vi "edge_detecting.vi"(0 "Image In":T5=refnum, 1 "mid_near Edge Options":T3={"Edge Polarity"=0, "Kernel Size"=3, "Width"=3, "Minimum Edge Strength"=10.0, "Interpolation Type"=enum."Bilinear Fixed", "Data Processing Method"=enum."Average"} {"Edge Polarity" items=["All Edges", "Rising Edges", "Falling Edges"]}, 2 "mid_far Edge Options":T3={"Edge Polarity"=0, "Kernel Size"=3, "Width"=3, "Minimum Edge Strength"=10.0, "Interpolation Type"=enum."Bilinear Fixed", "Data Processing Method"=enum."Average"} {"Edge Polarity" items=["All Edges", "Rising Edges", "Falling Edges"]}, 4 "mid_near Descriptor":T4={"Global Rectangle"=[276, 216, 344, 218], "Contours"=[{"ID"=enum."External", "Type"=2, "Coordinates"=[276, 216, 343, 217]}]} {"Contours"."Type" items=["No Selection", "Point", "Line", "Rectangle", "Oval", "Polygon", "Freehand Region", "Annulus", "Unused2", "Unused3", "Broken Line", "Freehand Line", "Rotated Rectangle"]}, 5 "mid_far Descriptor":T4={"Global Rectangle"=[475, 215, 533, 216], "Contours"=[{"ID"=enum."External", "Type"=2, "Coordinates"=[475, 215, 532, 215]}]} {"Contours"."Type" items=["No Selection", "Point", "Line", "Rectangle", "Oval", "Polygon", "Freehand Region", "Annulus", "Unused2", "Unused3", "Broken Line", "Freehand Line", "Rotated Rectangle"]}, 7 "error in":errorcluster) -> (20 "Image Out":T5, 21 "mid_near Edge Information":T1[](array[typedef]) {"Distance (Real-World)" format="%.2f"; "Location (Real-World)"."Y" format="%.2g"; "Location (Real-World)"."X" format="%.2f"; "Noise" format="%.2f"; "Location (Pixel)"."Y" format="%.2g"; "Location (Pixel)"."X" format="%.2f"; "Strength" format="%.2f"; "Distance (Pixel)" format="%.2f"}, 22 "mid_far Edge Information":T1[](array[typedef])=[{"Location (Pixel)"={"X"=519.67285, "Y"=215.0}, "Location (Real-World)"={"X"=240.41748, "Y"=115.199524}, "Distance (Pixel)"=44.6728401184082, "Distance (Real-World)"=30.526857895066314, "Strength"=12.0, "Noise"=4.0, "Rising?"=TRUE}] {"Distance (Real-World)" format="%.2f"; "Location (Real-World)"."Y" format="%.2g"; "Location (Real-World)"."X" format="%.2f"; "Noise" format="%.2f"; "Location (Pixel)"."Y" format="%.2g"; "Location (Pixel)"."X" format="%.2f"; "Strength" format="%.2f"; "Distance (Pixel)" format="%.2f"}, 25 "mid_near-edge_location":cluster{"X":sgl, "Y":sgl}[](array[cluster]), 26 "mid_far-edge_location":cluster{"X":sgl, "Y":sgl}[](array[cluster])=[{"X"=519.67285, "Y"=215.0}], 27 "error out":errorcluster)   [LabVIEW 2024]
uses:
  <vilib>/vision/Image Controls.llb/IMAQ Image.ctl
  <vilib>/vision/Measure.llb/Edge New.ctl
  <vilib>/vision/NI_Vision_Development_Module.lvlib
panel:
  in  "Process (Edge Detector mid_far)":T2(ring)=enum."Get First + Last Edge"
  in  "Process (Edge Detector mid_near)":T2(ring)=enum."Get First + Last Edge"
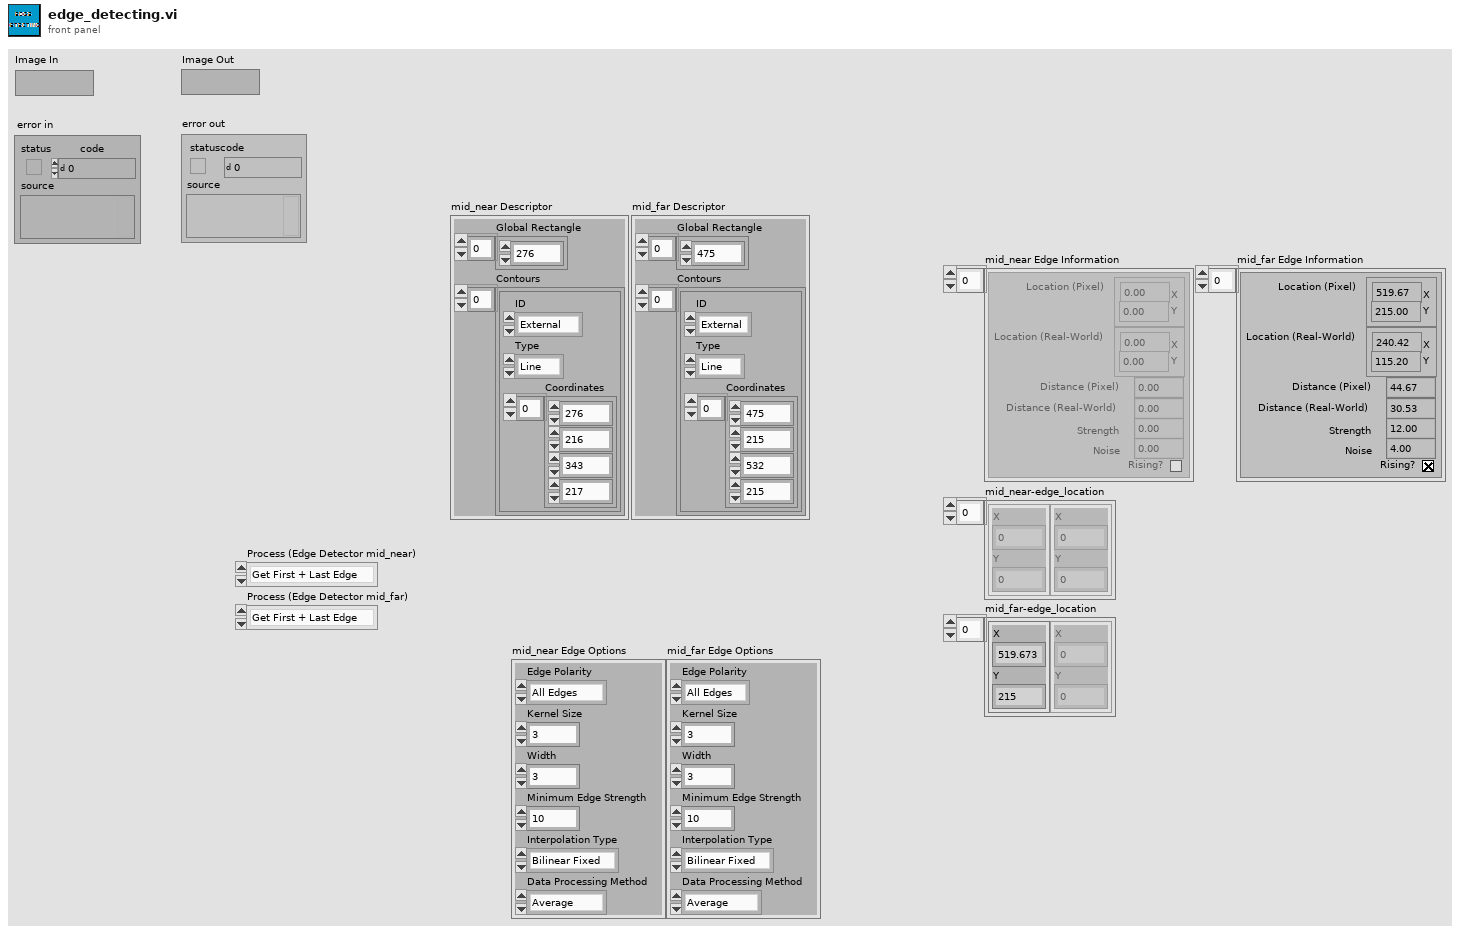
[diagram p1: front panel]
types:
  T1 = typedef "Edge New.ctl" = cluster{"Location (Pixel)":cluster{"X":sgl, "Y":sgl}, "Location (Real-World)":cluster{"X":sgl, "Y":sgl}, "Distance (Pixel)":dbl, "Distance (Real-World)":dbl, "Strength":dbl, "Noise":dbl, "Rising?":bool}
  T2 = enum16{"Get First Edge", "Get First + Last Edge", "Get All Edges", "Get Best Edge"}
  T3 = cluster{"Edge Polarity":u32, "Kernel Size":u32, "Width":u32, "Minimum Edge Strength":sgl, "Interpolation Type":enum32{"Zero Order", "Bilinear", "Quadratic", "Cubic", "Bilinear Fixed"}, "Data Processing Method":enum32{"Average", "Median"}}
  T4 = cluster{"Global Rectangle":i32[], "Contours":cluster{"ID":enum32{"External", "Internal"}, "Type":u32, "Coordinates":i32[]}[]}
  T5 = typedef "IMAQ Image.ctl" = refnum<image>
  T6 = cluster{"Origin Pixel":cluster{"X":sgl, "Y":sgl}, "X Axis Pixel":cluster{"X":sgl, "Y":sgl}, "Axis Reference":u32}
  T7 = cluster{"ID":enum32{"External", "Internal"}, "Type":u32, "Coordinates":i32[]}[]
  T8 = cluster{"ID":enum32{"External", "Internal"}, "Type":u32, "Coordinates":i32[]}
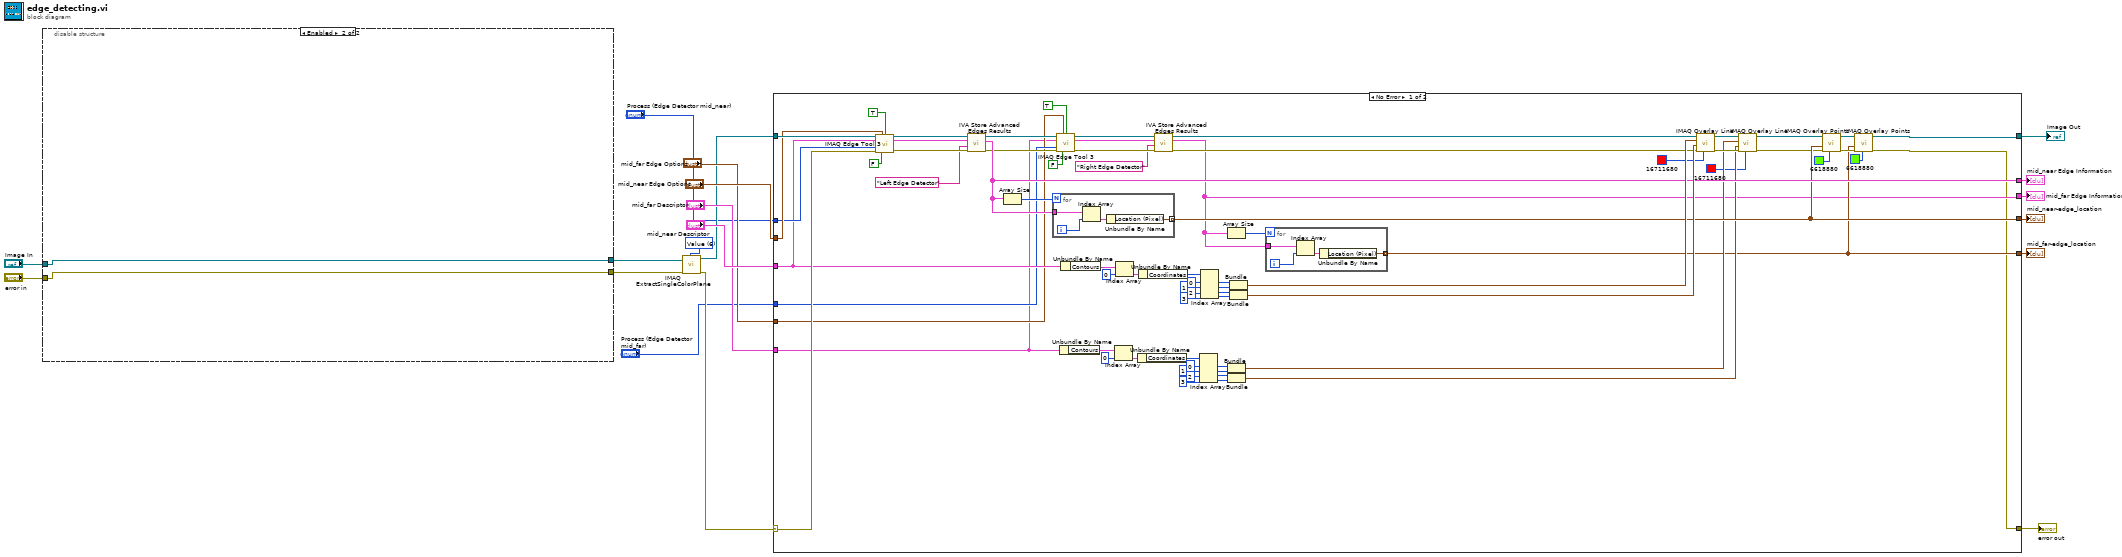
[diagram p0: block diagram]
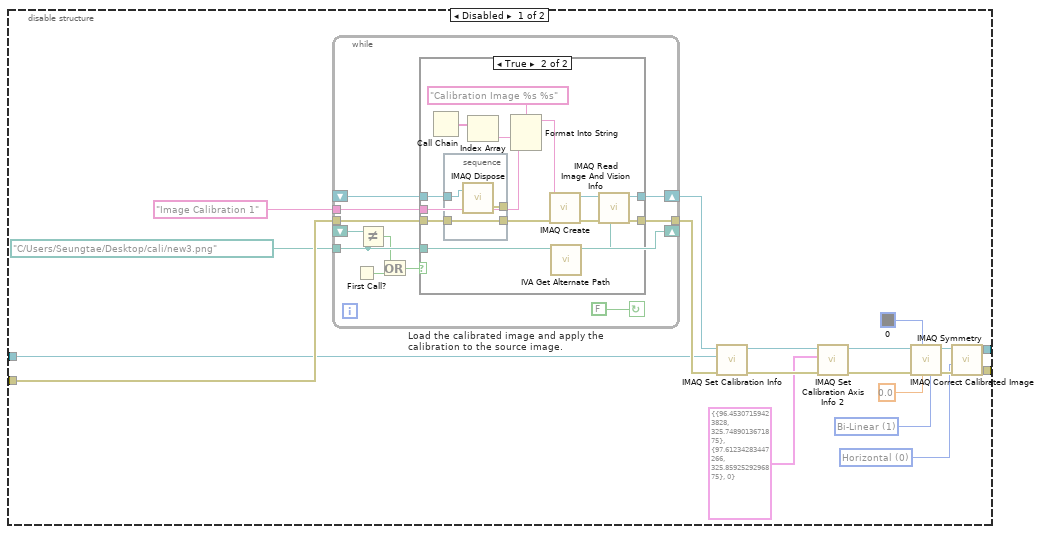
[diagram p2: hidden frame]
diagram:
  w16 = 6 items=["Red", "Green", "Blue", "Hue", "Saturation", "Luminance", "Value", "Intensity"] ("Color Plane")
  n1 = disable-structure shown="Enabled" {
    disable-tunnel: "error in" -> [w38 w69]
    disable-tunnel: "Image In" -> [w33 w70]
    disable-tunnel: [w22 w69] -> w17
    disable-tunnel: [w20 w70] -> w15
    frame Disabled {
      w21 = u32 0 items=["Horizontal", "Vertical", "Central", "1st Diagonal", "2nd Diagonal"] ("Type of Symmetry")
      w28 = u32 1 items=["Zero Order", "Bi-Linear", "Quadratic", "Cubic Spline"] ("Interpolation Type")
      n2 = while "Load the calibrated image and apply the calibration to the source image." {
        shift-right: [w49] -> w36
        shift-left: _ -> [w48]
        tunnel: [w46] -> w35
        tunnel: w38 -> [w45]
        tunnel: path "C:/Users/Seungtae/Desktop/cali/new3.png" ("File Path") -> [w42]
        tunnel: "Image Calibration 1" ("Step Name") -> [w44]
        shift-right: [w42] -> _
        shift-left: _ -> [w43]
        stop <- FALSE continue-if-true
        n3 = First Call?() -> (First Call?: T/F=w41:bool)
        n4 = Not Equal?(x=w43, y=w42) -> (x != y?=w40:bool)
        n5 = Or(x=w40, y=w41) -> (x .or. y?=w39:bool)
        n6 = case shown="True" w39 {
          tunnel: [w51 w63] -> w49
          tunnel: w48 -> [w51 w55]
          tunnel: [w50 w60] -> w46
          tunnel: w45 -> [w50 w56]
          tunnel: w42 -> [_ w53]
          tunnel: w44 -> [_ w57]
          frame False {
          }
          frame True {
            n7 = Call Chain() -> (call chain=w59:string[])
            n8 = stacked-sequence {
              tunnel: w56 -> [w67]
              tunnel: w55 -> [w68]
              tunnel: [w67] -> w54
              tunnel: [w66] -> _
              frame #0 {
                n9 = call "IMAQ Dispose"("Image"=w68) -> ("error out"=w66:errorcluster)  [unwired: 2 in, 3 out]
              }
            }
            n10 = Index Array(array=w59) -> (element=w58:string)  [unwired: 1 in]
            n11 = Format Into String(format string="Calibration Image %s %s" ("Image Name"), w58, w57) -> (resulting string=w65:string)  [unwired: 2 in, 1 out]
            n12 = call "IMAQ Create"("Image Name"=w65, "error in (no error)"=w54) -> ("New Image"=w62:T5, "error out"=w61:errorcluster)  [unwired: 2 in, 1 out]
            n13 = call <vilib>:"IVA Get Alternate Path.vi"("Path In"=w53) -> ("Path Out"=w52:path)  [unwired: 10 out]
            n14 = call "IMAQ Read Image And Vision Info"("File Path"=w52, "error in (no error)"=w61, "Image"=w62) -> ("error out"=w60:errorcluster, "Image Out"=w63:T5)  [unwired: 1 in, 6 out]
          }
        }
      }
      n15 = call "IMAQ Set Calibration Info"("error in (no error)"=w35, "Image Dst"=w33, "Image Src"=w36) -> ("error out"=w34:errorcluster, "Calibrated Image"=w30:T5)  [unwired: 1 in, 6 out]
      n16 = call-poly "IMAQ Set Calibration Axis Info 2"("error in (no error)"=w34, "Calibration Axis Info"=T6 {"Origin Pixel"={"X"=96.45307, "Y"=325.7489}, "X Axis Pixel"={"X"=97.61234, "Y"=325.85925}, "Axis Reference"=0}, "Calibration Template Image In"=w30) -> ("error out"=w31:errorcluster, "Calibration Template Image Out"=w26:T5)  [unwired: 7 out]
      n17 = call "IMAQ Correct Calibrated Image"("Interpolation Type"=w28, "Replace Value"=sgl 0.0, "Color Replace Value"=u32 0, "error in (no error)"=w31, "Image Src"=w26) -> ("error out"=w27:errorcluster, "Corrected Image"=w23:T5)  [unwired: 2 in, 3 out]
      n18 = call "IMAQ Symmetry"("error in (no error)"=w27, "Type of Symmetry"=w21, "Image Src"=w23) -> ("error out"=w22:errorcluster, "Image Dst Out"=w20:T5)  [unwired: 1 in, 1 out]
    }
    frame Enabled {
    }
  }
  n19 = call "IMAQ ExtractSingleColorPlane"("Color Plane"=w16, "error in (no error)"=w17, "Image Src"=w15) -> ("error out"=w9:errorcluster, "Image Dst Out"=w10:T5)  [unwired: 1 in, 6 out]
  n20 = case shown="No Error" w9 {
    selector: w9 -> [w137 w149]
    tunnel: w10 -> [w140 w150]
    tunnel: "mid_near Edge Options" -> [w134 _]
    tunnel: "mid_near Descriptor" -> [w117 _]
    tunnel: "Process (Edge Detector mid_near)" -> [w133 _]
    tunnel: [w72 w150] -> w6
    tunnel: [w71 w149] -> w5
    tunnel: [w112 _] -> w4
    tunnel: [w111 _] -> w2
    tunnel: "Process (Edge Detector mid_far)" -> [w106 _]
    tunnel: "mid_far Edge Options" -> [w105 _]
    tunnel: "mid_far Descriptor" -> [w88 _]
    tunnel: [w79 _] -> w1
    tunnel: [w73 _] -> w3
    frame No Error {
      n21 = call "IMAQ Edge Tool 3"("Image"=w140, "Edge Options"=w134, "Optimized Mode"=TRUE, "ROI Descriptor"=w117, "Process"=w133, "error in (no error)"=w137, "Reverse Direction"=FALSE) -> ("Image (duplicate)"=w139:T5, "Edge Information"=w136:T1[], "error out"=w138:errorcluster)  [unwired: 6 out]
      n22 = call <vilib>:"IVA Store Advanced Edges Results.vi"("error in (no error)"=w138, "Step Name"="Left Edge Detector", "Edge Information"=w136, "Image in"=w139) -> ("error out"=w109:errorcluster, "Edge Information dup"=w112:T1[], "Image dup"=w110:T5)  [unwired: 5 out]
      n23 = Array Size(array=w112) -> (size(s)=w130:i32)
      n24 = for {
        N: w130 -> [_]
        tunnel: w112 -> [w148]
        tunnel: [w145] -> w111 mode=indexing
        i -> [w147]
        n25 = Index Array(array=w148, index=w147) -> (element=w146:T1)
        n26 = Unbundle By Name(w146) -> ("Location (Pixel)"=w145:cluster{"X":sgl, "Y":sgl})
      }
      n27 = call "IMAQ Edge Tool 3"("Image"=w110, "Edge Options"=w105, "Optimized Mode"=TRUE, "ROI Descriptor"=w88, "Process"=w106, "error in (no error)"=w109, "Reverse Direction"=FALSE) -> ("Image (duplicate)"=w108:T5, "Edge Information"=w101:T1[], "error out"=w107:errorcluster)  [unwired: 6 out]
      n28 = Unbundle By Name(w88) -> ("Contours"=w99:T7)
      n29 = Unbundle By Name(w117) -> ("Contours"=w128:T7)
      n30 = Index Array(array=w99, index=0 ("인덱스")) -> (element=w98:T8)
      n31 = Index Array(array=w128, index=0 ("인덱스")) -> (element=w127:T8)
      n32 = Unbundle By Name(w98) -> ("Coordinates"=w97:i32[])
      n33 = Unbundle By Name(w127) -> ("Coordinates"=w126:i32[])
      n34 = call <vilib>:"IVA Store Advanced Edges Results.vi"("error in (no error)"=w107, "Step Name"="Right Edge Detector", "Edge Information"=w101, "Image in"=w108) -> ("error out"=w76:errorcluster, "Edge Information dup"=w73:T1[], "Image dup"=w77:T5)  [unwired: 5 out]
      n35 = Index Array(array=w97, index #1=0 ("인덱스"), index #2=1 ("인덱스"), index #3=2 ("인덱스"), index #4=3 ("인덱스")) -> (element #1=w92:i32, element #2=w91:i32, element #3=w90:i32, element #4=w89:i32)
      n36 = Index Array(array=w126, index #1=0 ("인덱스"), index #2=1 ("인덱스"), index #3=2 ("인덱스"), index #4=3 ("인덱스")) -> (element #1=w121:i32, element #2=w120:i32, element #3=w119:i32, element #4=w118:i32)
      n37 = Array Size(array=w73) -> (size(s)=w82:i32)
      n38 = Bundle(w92, w91) -> (w85:cluster{i32, i32})  [unwired: 1 in]
      n39 = Bundle(w90, w89) -> (w84:cluster{i32, i32})  [unwired: 1 in]
      n40 = Bundle(w121, w120) -> (w116:cluster{i32, i32})  [unwired: 1 in]
      n41 = Bundle(w119, w118) -> (w115:cluster{i32, i32})  [unwired: 1 in]
      n42 = for {
        N: w82 -> [_]
        tunnel: w73 -> [w144]
        tunnel: [w141] -> w79 mode=indexing
        i -> [w143]
        n43 = Index Array(array=w144, index=w143) -> (element=w142:T1)
        n44 = Unbundle By Name(w142) -> ("Location (Pixel)"=w141:cluster{"X":sgl, "Y":sgl})
      }
      n45 = call "IMAQ Overlay Line"("Color"=u32 16711680, "error in (no error)"=w76, "End Point"=w115, "Start Point"=w116, "Image"=w77) -> ("error out"=w86:errorcluster, "Image Out"=w87:T5)  [unwired: 5 in]
      n46 = call "IMAQ Overlay Line"("Color"=u32 16711680, "error in (no error)"=w86, "End Point"=w84, "Start Point"=w85, "Image"=w87) -> ("error out"=w74:errorcluster, "Image Out"=w75:T5)  [unwired: 5 in]
      n47 = call "IMAQ Overlay Points"("Color"=u32 6618880, "error in (no error)"=w74, "Array of Points"=w111, "Image"=w75) -> ("error out"=w81:errorcluster, "Image Out"=w80:T5)  [unwired: 6 in]
      n48 = call "IMAQ Overlay Points"("Color"=u32 6618880, "error in (no error)"=w81, "Array of Points"=w79, "Image"=w80) -> ("error out"=w71:errorcluster, "Image Out"=w72:T5)  [unwired: 6 in]
    }
    frame Error {
    }
  }
  "Image Out" <- w6
  "error out" <- w5
  "mid_near Edge Information" <- w4
  "mid_far Edge Information" <- w3
  "mid_near-edge_location" <- w2
  "mid_far-edge_location" <- w1
